vi "Alerte vide.vi"() -> ()   [LabVIEW 2022 SP3]
uses:
  Enum/Enum 2.ctl
  Variables globales/Variable glob alertes pressions.vi
  Variables globales/Variable glob Edwards.vi
  Variables globales/Variable glob Leybold.vi
panel:
  out "Nb pages":u8
  in  "ajouter":bool
  in  "Groupes":T1(array[cluster])=[{"valeur"=1e-05, "Alerte"=FALSE, "Pressions a surveiller :"=[], "N°"=0}] caption="Groupes alertes pressions" {"valeur" min=1e-07 max=1000.0 step=1e-07 format="%.2e"}
  in  "OK":bool
  in  "Annuler":bool
  # "PARAMETRES POUR\nALERTE PRESSION PAR ENVOI D'UN MAIL"
  # "Ce logiciel et les informations qu'il contient, sont la propriété de l’IAS et ne peuvent être diffusés sans l’autorisation de la Station d’étalonnage"
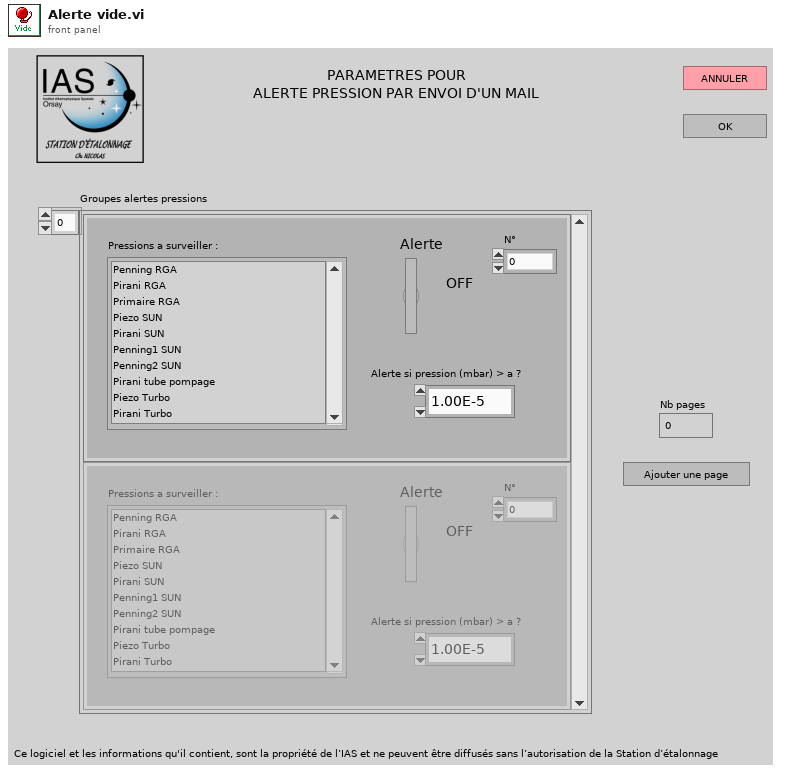
[diagram p1: front panel]
types:
  T1 = cluster{"valeur":dbl, "Alerte":bool, "Pressions a surveiller :":i32[], "N°":u16}[]
  T2 = typedef "Enum 2.ctl" = enum16{"init noms", "initialisation", "choix", "GO"}
  T3 = cluster{"Alerte":bool, "valeur ":dbl, "Défaut":bool, "Indices controler":i16[], "N°":u16}[]
  T4 = cluster{"valeur":dbl, "Alerte":bool, "Pressions a surveiller :":i32[], "N°":u16}
  T5 = cluster{"Alerte":bool, "valeur ":dbl, "Défaut":bool, "Indices controler":i16[], "N°":u16}
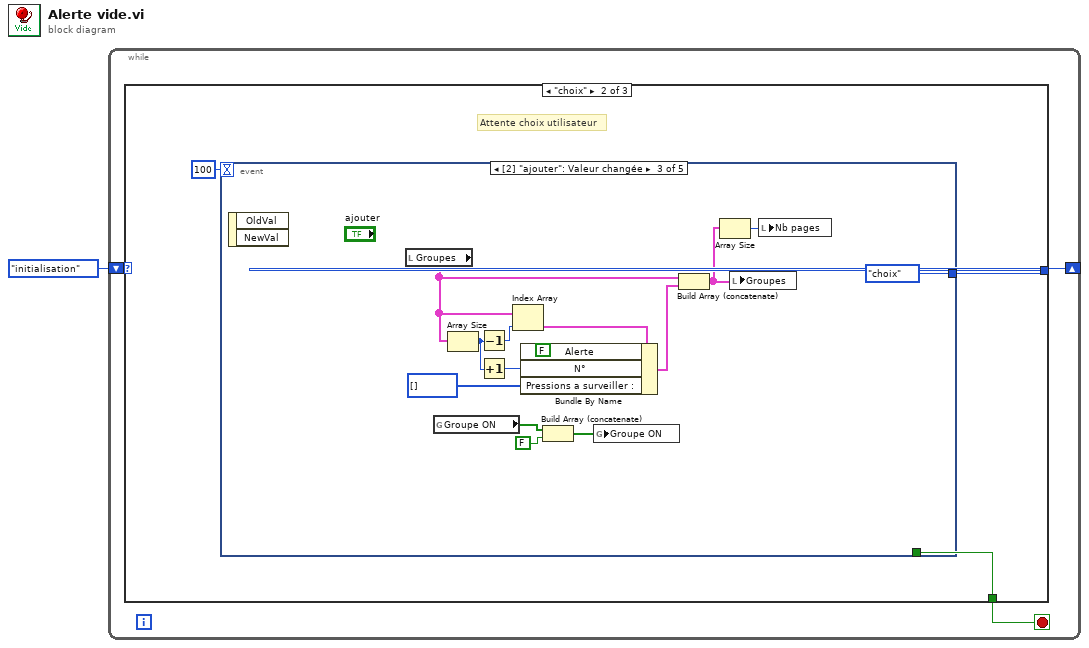
[diagram p0: block diagram]
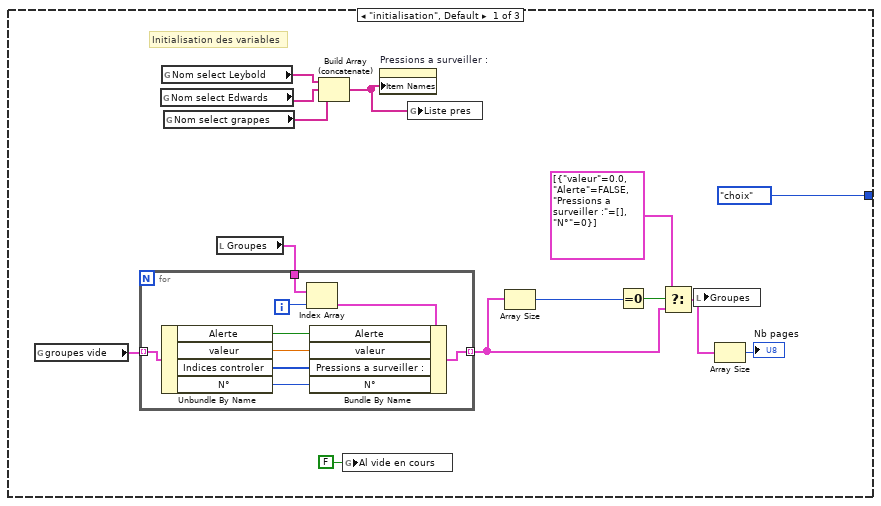
[diagram p2: hidden frame]
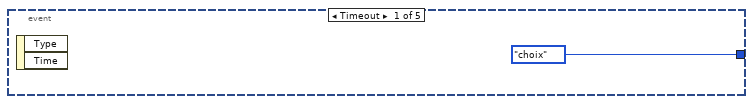
[diagram p3: hidden frame]
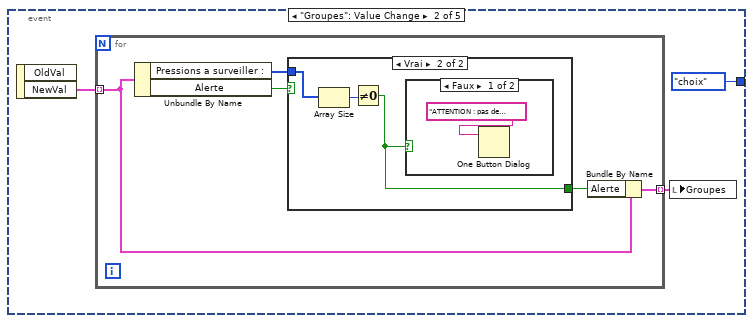
[diagram p4: hidden frame]
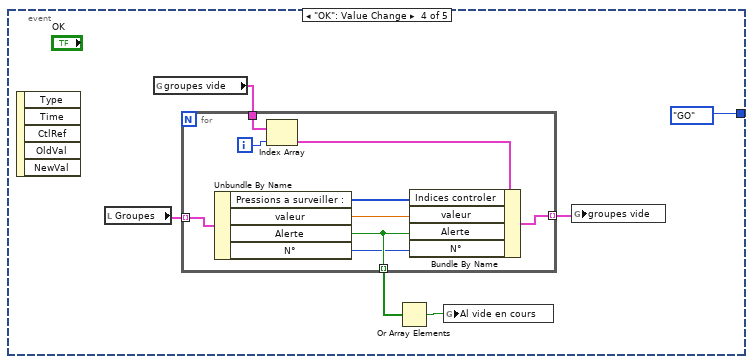
[diagram p7: hidden frame]
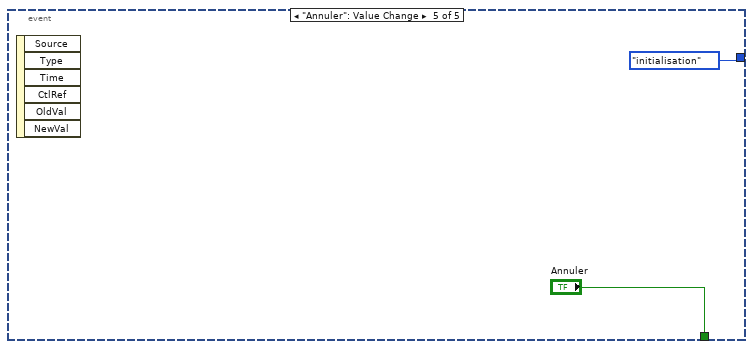
[diagram p8: hidden frame]
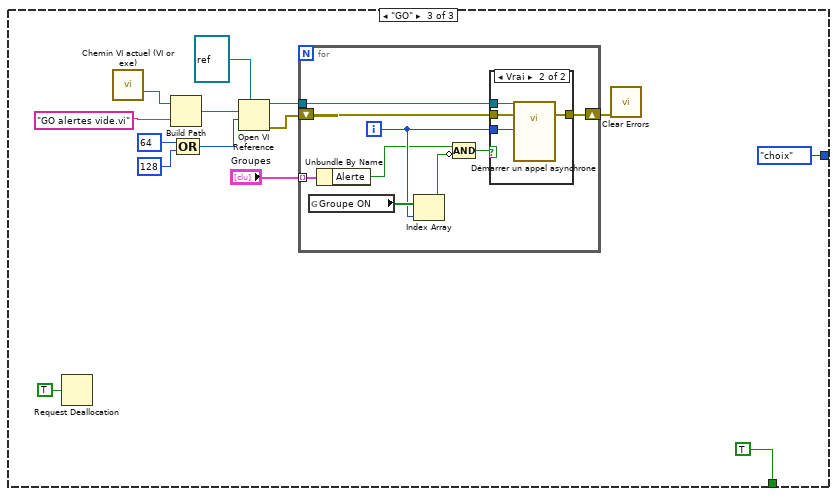
[diagram p9: hidden frame]
diagram:
  n1 = while {
    shift-right: [w3] -> _
    shift-left: Enum_2."initialisation" ("Énum") -> [w4]
    stop <- w2 stop-if-true
    n2 = case shown="\"choix\"" w4 {
      tunnel: [Enum_2."choix" ("Énum") w29 Enum_2."choix" ("Énum")] -> w3
      tunnel: [_ w28 TRUE] -> w2
      frame "initialisation", Default {
        # "Initialisation des variables"
        n3 = global read "Variable glob alertes pressions.vi" "groupes vide"() -> (w15:T3)
        n4 = global read "Variable glob Edwards.vi" "Nom select Edwards"() -> (w18:string[])
        n5 = global read "Variable glob Leybold.vi" "Nom select Leybold"() -> (w17:string[])
        n6 = global read "Variable glob Edwards.vi" "Nom select grappes"() -> (w11:string[])
        n7 = local read "Groupes"() -> (w14:T1)
        n8 = for {
          tunnel: w15 -> [w27] mode=indexing
          tunnel: w14 -> [w26]
          tunnel: [w21] -> w8 mode=indexing
          i -> [w20]
          n9 = Unbundle By Name(w27) -> ("Alerte"=w22:bool, "valeur"=w24:dbl, "Indices controler"=w23:i16[], "N°"=w19:u16)
          n10 = Index Array(array=w26, index=w20) -> (element=w25:T4)
          n11 = Bundle By Name(cluster=w25, "Alerte"=w22, "valeur"=w24, "Pressions a surveiller :"=w23, "N°"=w19) -> (w21:T4)
        }
        n12 = Build Array (concatenate)(w17, w18, w11) -> (w12:string[])
        n13 = global write "Variable glob alertes pressions.vi" "Al vide en cours"(FALSE ("Al vide en cours")) -> ()
        n14 = property on="Pressions a surveiller :" class="LstDér (strict)"("Item Names"=w12) -> ()  [unwired: 2 in, 2 out]
        n15 = global write "Variable glob alertes pressions.vi" "Liste pres"(w12) -> ()
        n16 = Array Size(array=w8) -> (size(s)=w9:i32)
        n17 = Equal To 0?(x=w9) -> (x = 0?=w10:bool)
        n18 = Select(t=T1 [{"valeur"=0.0, "Alerte"=FALSE, "Pressions a surveiller :"=[], "N°"=0}] ("cas vrai"), s=w10, f=w8) -> (s? t:f=w6:T1)
        n19 = local write "Groupes"(w6) -> ()
        n20 = Array Size(array=w6) -> (size(s)=→"Nb pages":i32)
      }
      frame "choix" {
        # "Attente choix utilisateur"
        n21 = event shown="[2] \"ajouter\": Valeur changée" {
          selector: _ -> [_ _ _ _ _]
          dyn-events: _ -> [_ _ _ _ _]
          timeout: 100 -> [_ _ _ _ _]
          tunnel: [Enum_2."choix" ("Énum") Enum_2."choix" ("Énum") Enum_2."choix" ("Énum") Enum_2."GO" ("Énum") Enum_2."initialisation" ("Énum")] -> w29
          tunnel: [_ _ _ _ "Annuler"] -> w28
          event Timeout {
            n22 = event-data() -> ()  [unwired: 1 in, 2 out]
          }
          event "Groupes": Value Change {
            n23 = event-data() -> ("NewVal"=w34:T1)  [unwired: 1 in, 1 out]
            n24 = for {
              tunnel: w34 -> [w38] mode=indexing
              tunnel: [w35] -> w33 mode=indexing
              n25 = Unbundle By Name(w38) -> ("Pressions a surveiller :"=w37:i32[], "Alerte"=w39:bool)
              n26 = case shown="Vrai" w39 {
                selector: w39 -> [w40 _]
                tunnel: w37 -> [_ w43]
                tunnel: [w40 w41] -> w36
                frame False {
                }
                frame True {
                  n27 = Array Size(array=w43) -> (size(s)=w42:i32)
                  n28 = Not Equal To 0?(x=w42) -> (x != 0?=w41:bool)
                  n29 = case shown="Faux" w41 {
                    frame False {
                      n30 = One Button Dialog(message="ATTENTION : pas de capteur choisi dans la liste") -> ()  [unwired: 1 in, 1 out]
                    }
                    frame True {
                    }
                  }
                }
              }
              n31 = Bundle By Name(cluster=w38, "Alerte"=w36) -> (w35:T4)
            }
            n32 = local write "Groupes"(w33) -> ()
          }
          event "ajouter": Value Change {
            n33 = event-data() -> ()  [unwired: 1 in, 2 out]
            n34 = local read "Groupes"() -> (w56:T1)
            n35 = global read "Variable glob alertes pressions.vi" "Groupe ON"() -> (w50:bool[])
            n36 = Array Size(array=w56) -> (size(s)=w47:i32)
            n37 = Decrement(x=w47) -> (x-1=w57:i32)
            n38 = Increment(x=w47) -> (x+1=w46:i32)
            n39 = Index Array(array=w56, index=w57) -> (element=w55:T4)
            n40 = Bundle By Name(cluster=w55, "Alerte"=FALSE, "N°"=w46, "Pressions a surveiller :"=i32[] []) -> (w53:T4)
            n41 = Build Array (concatenate)(w50, FALSE) -> (w48:bool[])
            n42 = global write "Variable glob alertes pressions.vi" "Groupe ON"(w48) -> ()
            n43 = Build Array (concatenate)(w56, w53) -> (w52:T1)
            n44 = Array Size(array=w52) -> (size(s)=w51:i32)
            n45 = local write "Groupes"(w52) -> ()
            n46 = local write "Nb pages"(w51) -> ()
          }
          event "OK": Value Change {
            n47 = event-data() -> ()  [unwired: 1 in, 5 out]
            n48 = local read "Groupes"() -> (w64:T1)
            n49 = global read "Variable glob alertes pressions.vi" "groupes vide"() -> (w63:T3)
            n50 = for {
              tunnel: w64 -> [w73] mode=indexing
              tunnel: w63 -> [w72]
              tunnel: [w67] -> w62 mode=indexing
              tunnel: [w66] -> w61 mode=indexing
              i -> [w71]
              n51 = Unbundle By Name(w73) -> ("Pressions a surveiller :"=w69:i32[], "valeur"=w68:dbl, "Alerte"=w66:bool, "N°"=w65:u16)
              n52 = Index Array(array=w72, index=w71) -> (element=w70:T5)
              n53 = Bundle By Name(cluster=w70, "Indices controler"=w69, "valeur"=w68, "Alerte"=w66, "N°"=w65) -> (w67:T5)
            }
            n54 = Or Array Elements(Boolean array=w61) -> (logical OR=w60:bool)
            n55 = global write "Variable glob alertes pressions.vi" "Al vide en cours"(w60) -> ()
            n56 = global write "Variable glob alertes pressions.vi" "groupes vide"(w62) -> ()
          }
          event "Annuler": Value Change {
            n57 = event-data() -> ()  [unwired: 1 in, 6 out]
          }
        }
      }
      frame "GO" {
        n58 = Request Deallocation(TRUE ("flag")) -> ()
        n59 = call "Chemin VI actuel (VI or exe).vi"() -> ("VI or executable installation directory"=w82:path)  [unwired: 14 in, 1 out]
        n60 = Build Path(base path=w82, name or relative path="GO alertes vide.vi" ("nom ou chemin relatif")) -> (appended path=w86:path)
        n61 = Compound Arithmetic op=OR(64 ("options"), 128 ("options")) -> (w83:i32)
        n62 = Open VI Reference(type specifier VI Refnum (for type only)=refnum<vi> refnum ("spécificateur de type du refnum de VI (pour type seulement)"), vi path=w86, options=w83) -> (vi reference=w81:refnum<vi>, error out=w80:errorcluster)  [unwired: 3 in]
        n63 = for {
          shift-right: [w97] -> w78
          shift-left: w80 -> [w98]
          tunnel: w81 -> [w96]
          tunnel: "Groupes" -> [w95] mode=indexing
          i -> [w93]
          n64 = global read "Variable glob alertes pressions.vi" "Groupe ON"() -> (w94:bool[])
          n65 = Unbundle By Name(w95) -> ("Alerte"=w92:bool)
          n66 = Index Array(array=w94, index=w93) -> (element=w91:bool)
          n67 = Compound Arithmetic op=AND ("Opérateur arithmétique")(w92, invert w91) -> (w90:bool)
          n68 = case shown="Vrai" w90 {
            tunnel: w98 -> [w99 w103]
            tunnel: [w99 w102] -> w97
            tunnel: w96 -> [_ w101]
            tunnel: w93 -> [_ w100]
            frame False {
            }
            frame True {
              n69 = call-by-ref "Démarrer un appel asynchrone"(reference=w101, error in=w103, "Numéro"=w100) -> (error out=w102:errorcluster)  [unwired: 5 in, 1 out]
            }
          }
        }
        n70 = call <vilib>:"Clear Errors.vi"("error in (no error)"=w78) -> ()  [unwired: 5 in, 2 out]
      }
    }
  }
